vi "Labo03_PT100.vi"() -> ()   [LabVIEW 2021]
uses:
  <instrlib>/Agilent 3446X Series/Public/Data/Read (Multiple Points).vi
  <instrlib>/Agilent 3446X Series/Agilent 3446X Series.lvlib
panel:
  out "Waveform Chart":dbl[](graph)
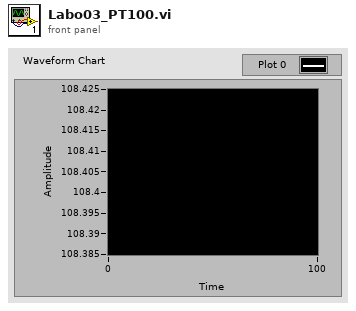
[diagram p1: front panel]
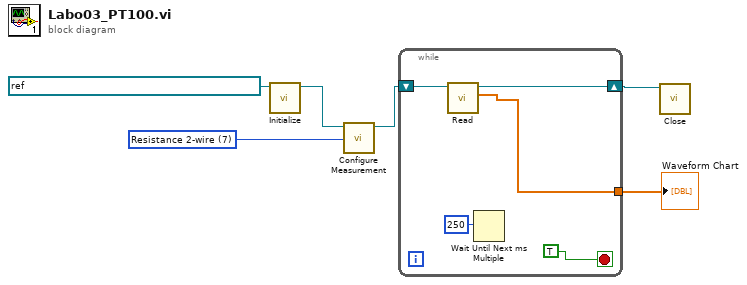
[diagram p0: block diagram]
diagram:
  w2 = 7 items=["Continuity", "Current AC", "Current DC", "Diode", "Frequency", "Resistance 4-wire", "Period", "Resistance 2-wire", "Temperature", "Voltage AC", "Voltage DC", "Voltage DC Ratio", "Capacitance"] ("Measurement Function (10: Voltage DC)")
  n1 = call <instrlib>:"Initialize.vi"("VISA resource name"=refnum<visa-resource-name> "USB0::0x2A8D::0x1601::MY53102179::INSTR") -> ("VISA resource name out"=w4:refnum<visa-resource-name>)  [unwired: 9 in, 1 out]
  n2 = call <instrlib>:"Configure Measurement.vi"("Measurement Function (10: Voltage DC)"=w2, "VISA resource name"=w4) -> ("VISA resource name out"=w5:refnum<visa-resource-name>)  [unwired: 8 in, 1 out]
  n3 = while {
    shift-right: [w11] -> w6
    shift-left: w5 -> [w10]
    tunnel: [w7] -> w1
    stop <- TRUE stop-if-true
    n4 = call-poly <instrlib>:"Read.vi"("VISA resource name"=w10) -> ("Measurements"=w7:dbl[], "VISA resource name out"=w11:refnum<visa-resource-name>)  [unwired: 8 in, 1 out]
    n5 = Wait Until Next ms Multiple(millisecond multiple=250) -> ()  [unwired: 1 out]
  }
  "Waveform Chart" <- w1
  n6 = call <instrlib>:"Close.vi"("VISA resource name"=w6) -> ()  [unwired: 10 in, 1 out]
